vi "ConstructAuthority.vi"(8 "password":string, 9 "username":string, 10 "port":string, 11 "host":string) -> (3 "authority":string)   [LabVIEW 2013, in "openURI.lvlib"]
uses:
  openURI.lvlib
  isHEXDigit.vi
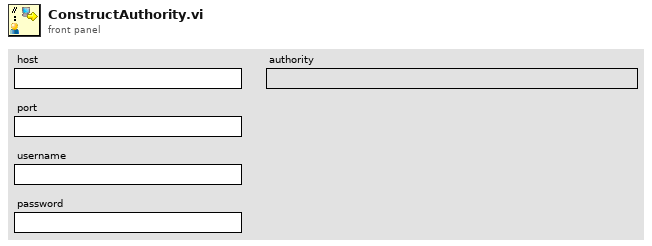
[diagram p1: front panel]
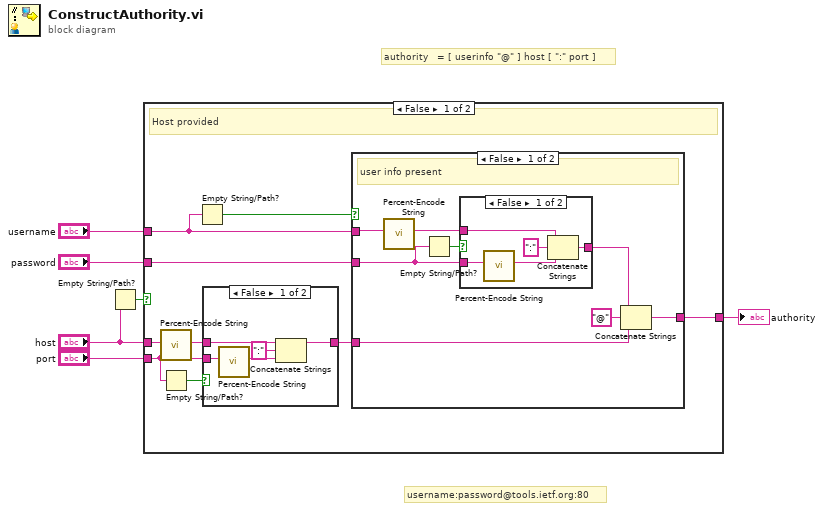
[diagram p0: block diagram]
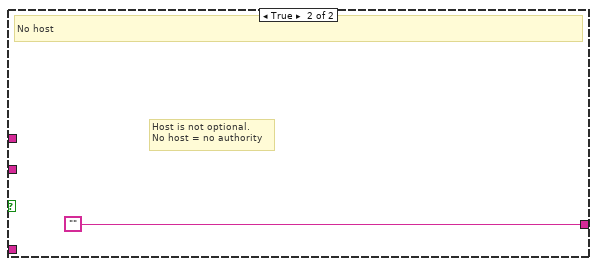
[diagram p5: hidden frame]
diagram:
  # "username:password@tools.ietf.org:80"
  # "authority   = [ userinfo \"@\" ] host [ \":\" port ]"
  n1 = Empty String/Path?(string/path="host") -> (empty?=w3:bool)
  n2 = case shown="False" w3 {
    tunnel: "username" -> [w14 _]
    tunnel: "password" -> [w13 _]
    tunnel: [w12 ""] -> w4
    tunnel: "host" -> [w8 _]
    tunnel: "port" -> [w10 _]
    frame False {
      # "Host provided"
      n3 = call "Percent-Encode String.vi"("String"=w8) -> ("Pct-Encoded String"=w7:string)  [unwired: 10 in]
      n4 = Empty String/Path?(string/path=w10) -> (empty?=w11:bool)
      n5 = Empty String/Path?(string/path=w14) -> (empty?=w15:bool)
      n6 = case shown="False" w11 {
        tunnel: w10 -> [w17 _]
        tunnel: [w19 w21] -> w9
        tunnel: w7 -> [w18 w21]
        frame False {
          n7 = call "Percent-Encode String.vi"("String"=w17) -> ("Pct-Encoded String"=w16:string)  [unwired: 10 in]
          n8 = Concatenate Strings(w18, ":" ("string"), w16) -> (w19:string)
        }
        frame True {
          # "No port"
        }
      }
      n9 = case shown="False" w15 {
        tunnel: w14 -> [w23 _]
        tunnel: w13 -> [w24 _]
        tunnel: [w28 w36] -> w12
        tunnel: w9 -> [w27 w36]
        frame False {
          # "user info present"
          n10 = call "Percent-Encode String.vi"("String"=w23) -> ("Pct-Encoded String"=w22:string)  [unwired: 10 in]
          n11 = Empty String/Path?(string/path=w24) -> (empty?=w25:bool)
          n12 = case shown="False" w25 {
            tunnel: w22 -> [w33 w35]
            tunnel: w24 -> [w31 _]
            tunnel: [w32 w35] -> w26
            frame False {
              n13 = call "Percent-Encode String.vi"("String"=w31) -> ("Pct-Encoded String"=w30:string)  [unwired: 10 in]
              n14 = Concatenate Strings(w33, ":" ("string"), w30) -> (w32:string)
            }
            frame True {
            }
          }
          n15 = Concatenate Strings(w26, "@" ("string"), w27) -> (w28:string)
        }
        frame True {
          # "No userinfo"
        }
      }
    }
    frame True {
      # "Host is not optional.\nNo host = no authority"
      # "No host"
    }
  }
  "authority" <- w4
